vi "DIALOG_Cluster Item Selection.vi"(7 "Action":T4=enum."Bundler Insert", 8 "Error In":errorcluster, 9 "User VI Ref":refnum<vi>, 10 "Affected Items":T2, 11 "Display Items":T3[](array[typedef])) -> (0 "Error Out":errorcluster, 1 "Hide Full Names Out":bool=TRUE, 2 "Action Choice Out":enum32{"Choice 1", "Choice 2"}(radio), 3 "Selected Items (tags)":string[](array[string]))   [LabVIEW 2023]
doc: "Dialog to select items from the input cluster ref. \n\nFilter narrows list of items.\nDown key puts focus on tree and selects first item.\nUp and Down keps navigate tree.\nMultiple items can be selected.\n\nIn case of action \"Delete\" (\"Remove elements(s)...\" selected), list will show all elements currently displayed, else it will show all elements availabel to undle or unbundle.\n\nOutput is a list of the selected item tags.\n\nSelected element is the item clicked in a bundler node, displayed ot help user remember where an insert will happen."
uses:
  controls/Done Button.ctl
  controls/action enum.ctl
  cluster/Cluster Element Description.ctl
  top/BundleMagic.ctl
  utils/Controls/Get-Set Enum.ctl
  LabVIEW-common/String/Select All/String Select All CTRL-A_all string.vi
  <userlib>/_OpenG.lib/appcontrol/appcontrol.llb/openg_application_control.lvlib
  <userlib>/_OpenG.lib/error/error.llb/openg_error.lvlib
  Libraries/Tree Handler/Tree Handlr.lvlib
panel:
  in  "Filter":string
  in  "Tree":string[](tree)
  in  "Hide Full Names":bool=TRUE
  in  "Select Unwired":bool
  out "Selected Element String":string
  in  "Action Choice Radio Buttons":enum32{"Choice 1", "Choice 2"}(radio)
  in  "Done":T1
  out "error out":errorcluster
  in  "Show radio":bool
  in  "C1":T5
  # "All panes scroll to origin at runtime, so we don't have to worry about pane placements\n\nThis pane contracts at runtime and vertical splitter to left sticks to right at runtime so resizing functions happen as expected."
  # "Debug"
  # "Debug Cluster"
  # "(Use for debug if display items empty)"
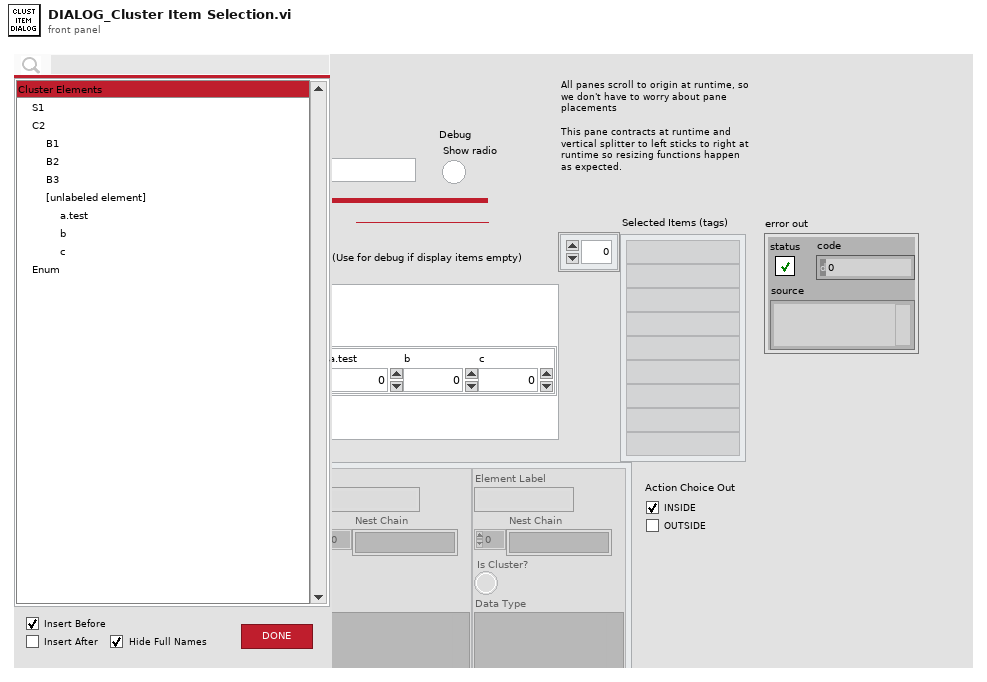
[diagram p1: front panel]
types:
  T1 = typedef "Done Button.ctl" = bool
  T2 = typedef "BundleMagic.ctl" = cluster{"Terminals":refnum<vi>[], "Wires":refnum<vi>[], "Named Bundler":refnum<vi>[], "Named Unbundler":refnum<vi>[], "In Place Cluster Node":refnum<vi>[], "Class Specifier Constant":refnum<vi>[], "Property Node":refnum<vi>[], "Invoke Node":refnum<vi>[], "Refnum Control":refnum<vi>[]}
  T3 = typedef "Cluster Element Description.ctl" = cluster{"Element Label":string, "Nest Chain":string[], "Is Cluster?":bool, "Data Type":variant, "Bundler Label":string, "Disabled":bool, "Unwired":bool, "Tree Tag":string}
  T4 = typedef "action enum.ctl" = enum16{"[NONE]", "APP_SEPARATOR", "Wire Bundle", "Wire Unbundle", "Terminal Unbundle", "Terminal Bundle", "Bundler Move Up", "Bundler Move Down", "Bundler Insert", "Bundler Remove", "Bundler Remove Unwired", "Bundler Reorder", "In Place Insert", "In Place Remove", "In Place Remove Unwired", "In Place Reorder", "Wire Properties", "Wire Method", "Terminal Properties", "Terminal Method", "Property Move Up", "Property Move Down", "Properties Insert", "Properties Remove", "Properties Remove Unwired", "Properties Reorder", "Method Change", "Class For Constant", "Class For Control", "Class For Node", "Class Name to Clipboard"}
  T5 = cluster{"S1":string, "C2":cluster{"B1":bool, "B2":bool, "B3":bool, cluster{"a.test":dbl, "b":i32, "c":u8}}, "Enum":enum16{""}}
  T6 = typedef "Get-Set Enum.ctl" = enum16{"Get", "Set"}
  T7 = typedef "LVPoint32TypeDef.ctl" = cluster{"Horizontal":i32, "Vertical":i32}
  T8 = cluster{"Shift":bool, "Ctrl":bool, "Alt":bool, "Cmd":bool, "Opt":bool}
  T9 = typedef "eventvkey.ctl" = enum16{"ASCII", "Enter", "Return", "Shift", "Ctrl", "Alt", "Cmd", "Opt", "Caps", "NumLock", "Clear", "Break", "Up", "Down", "Left", "Right", "Insert", "Delete", "Home", "End", "PageUp", "PageDown", "Escape", "Help", "Pause", "ScrollLock", "F1", "F2", "F3", "F4", "F5", "F6", "F7", "F8", "F9", "F10", "F11", "F12", "F13", "F14", "F15", "F16", "F17", "F18", "F19", "F20", "F21", "F22", "F23", "F24", "Play", "VolumeUp", "VolumeDown", "Mute", "Two Byte Char"}
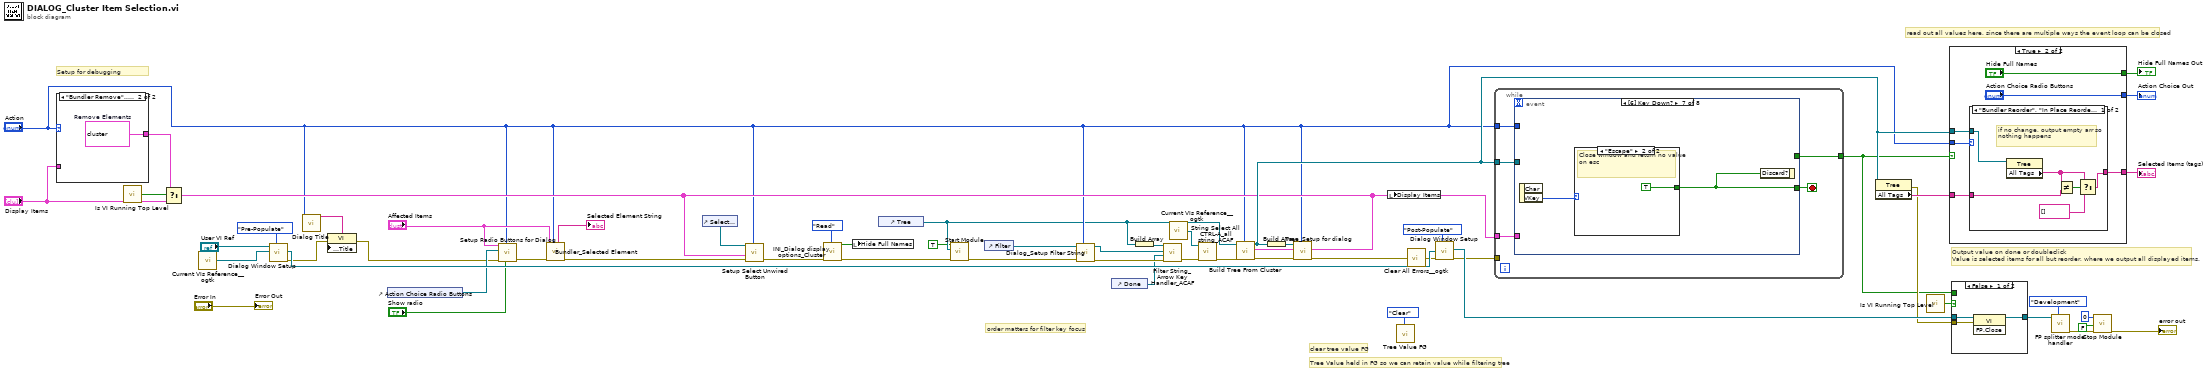
[diagram p0: block diagram]
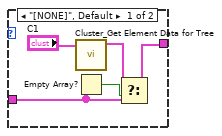
[diagram p2: hidden frame]
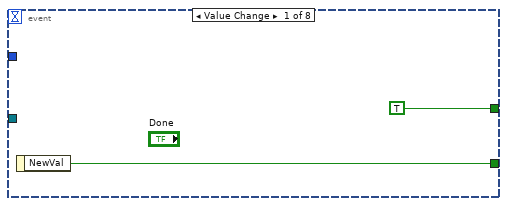
[diagram p3: hidden frame]
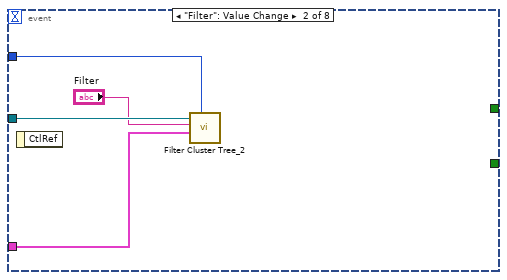
[diagram p4: hidden frame]
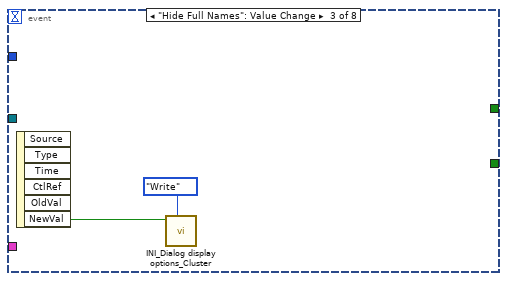
[diagram p5: hidden frame]
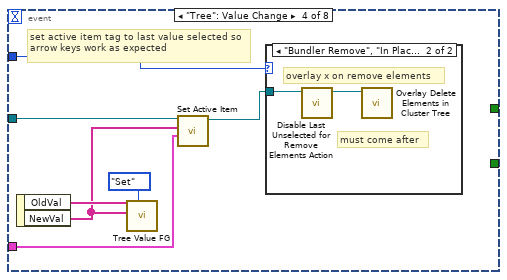
[diagram p6: hidden frame]
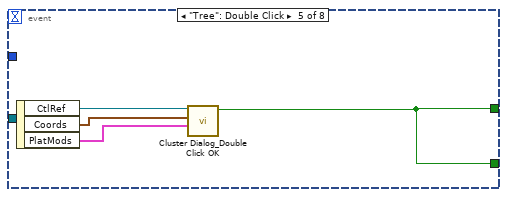
[diagram p8: hidden frame]
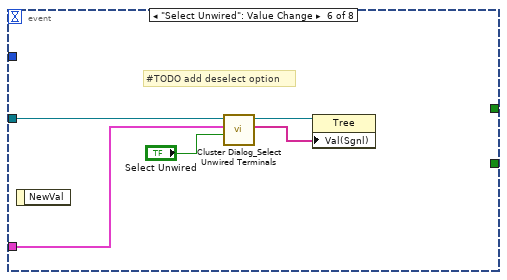
[diagram p9: hidden frame]
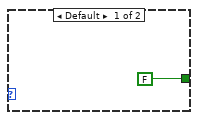
[diagram p10: hidden frame]
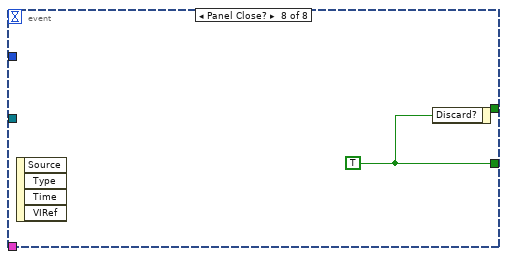
[diagram p11: hidden frame]
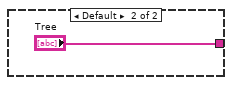
[diagram p13: hidden frame]
diagram:
  # "order matters for filter key focus"
  # "clear tree value FG"
  # "Setup for debugging"
  # "Tree Value held in FG so we can retain value while filtering tree"
  # "read out all values here, since there are multiple ways the event loop can be closed"
  # "Output value on done or doubleclick\nValue is selected items for all but reorder, where we output all displayed items."
  n1 = case shown="\"Bundler Remove\"..\"Bundler Reorder\"" "Action" {
    tunnel: [w61 w63] -> w46
    tunnel: "Display Items" -> [w60 _]
    frame "[NONE]", Default {
      n2 = call "Cluster_Get Element Data for Tree.vi"("Data Type"="C1") -> ("Cluster Element Data Aray"=w62:T3[])  [unwired: 10 in]
      n3 = Empty Array?(array=w60) -> (empty?=w59:bool)
      n4 = Select(t=w62, s=w59, f=w60) -> (s? t:f=w61:T3[])
    }
    frame "Bundler Remove".."Bundler Reorder" {
      w63 = T3[] [{"Element Label"="N1", "Nest Chain"=[], "Is Cluster?"=FALSE, "Data Type"=variant(dbl 0.0), "Bundler Label"="N1", "Disabled"=FALSE, "Unwired"=FALSE, "Tree Tag"="0[$`~g;}N1"}, {"Element Label"="N2", "Nest Chain"=["C1"], "Is Cluster?"=TRUE, "Data Type"=variant(dbl 0.0), "Bundler Label"="C1.N2", "Disabled"=FALSE, "Unwired"=FALSE, "Tree Tag"="C1[$`~g;}C1[$`~g;}N2"}, {"Element Label"="Boolean", "Nest Chain"=["C1"], "Is Cluster?"=TRUE, "Data Type"=variant(bool FALSE), "Bundler Label"="C1.Boolean", "Disabled"=FALSE, "Unwired"=TRUE, "Tree Tag"="C2[$`~g;}C1[$`~g;}Boolean"}, {"Element Label"="C1", "Nest Chain"=[], "Is Cluster?"=FALSE, "Data Type"=variant(cluster{"N2":dbl, "Boolean":bool} {"N2"=0.0, "Boolean"=FALSE}), "Bundler Label"="C1", "Disabled"=FALSE, "Unwired"=FALSE, "Tree Tag"="3[$`~g;}C1"}, {"Element Label"="String", "Nest Chain"=[], "Is Cluster?"=FALSE, "Data Type"=variant(string ""), "Bundler Label"="String", "Disabled"=FALSE, "Unwired"=FALSE, "Tree Tag"="4[$`~g;}String"}]  # Remove Elements
    }
  }
  n5 = call "Is VI Running Top Level.vi"() -> ("Top Level?"=w47:bool)  [unwired: 5 in]
  n6 = Select(t=w46, s=w47, f="Display Items") -> (s? t:f=w19:T3[])
  n7 = call <userlib>:"Current VIs Reference__ogtk.vi"() -> ("Current VI's reference"=w26:refnum<vi>)  [unwired: 5 in]
  n8 = call "Dialog Window Setup.vi"("Action"=enum16{"Pre-Populate", "Post-Populate"}."Pre-Populate", "Dialog VI Ref In [Parent]"=w26, "Align-to Window Ref"="User VI Ref") -> ("error out"=w24:errorcluster, "Dialog VI Ref Out"=w51:refnum<vi>)  [unwired: 7 in]
  n9 = call "Dialog Title.vi"("Action"="Action") -> ("Window Title"=w32:string)  [unwired: 10 in]
  n10 = property class="VI"(error in=w24, "Front Panel.Title"=w32) -> (error out=w23:errorcluster)  [unwired: 1 in, 1 out]
  n11 = control-ref of="Action Choice Radio Buttons"() -> (w34:refnum<vi>)
  n12 = call "Setup Radio Buttons for Dialog.vi"("Show Radio"="Show radio", "Action"="Action", "error in (no error)"=w23, "Action Choice Ref"=w34, "Affected Items"="Affected Items") -> ("error out"=w22:errorcluster)  [unwired: 6 in]
  n13 = call "Bundler_Selected Element.vi"("Action"="Action", "error in (no error)"=w22, "Affected Items"="Affected Items") -> ("error out"=w21:errorcluster, "Display String"=→"Selected Element String":string)  [unwired: 2 in, 5 out]
  n14 = control-ref of="Select Unwired"() -> (w33:refnum<vi>)
  n15 = call "Setup Select Unwired Button.vi"("Action"="Action", "error in (no error)"=w21, "Display Items"=w19, "Boolean in"=w33) -> ("error out"=w11:errorcluster)  [unwired: 7 in]
  n16 = call "INI_Dialog display options_Cluster.vi"("File Action"=enum16{"Read", "Write"}."Read", "error in (no error)"=w11) -> ("error out"=w6:errorcluster, "Hide Full Names Out"=w10:bool)  [unwired: 8 in]
  n17 = local write "Hide Full Names"(w10) -> ()
  n18 = control-ref of="Tree"() -> (w4:refnum<vi>)
  n19 = call "Start Module.vi"("error in"=w6, "Tree Ref"=w4, "Run as Singleton? (F)"=TRUE) -> ("error out"=w5:errorcluster)  [unwired: 5 in, 3 out]
  n20 = control-ref of="Filter"() -> (w27:refnum<vi>)
  n21 = call "Dialog_Setup Filter String.vi"("Action"="Action", "error in"=w5, "Filter String Ref"=w27) -> ("error out"=w18:errorcluster, "Filter String Ref Out"=w14:refnum<vi>)  [unwired: 7 in]
  n22 = control-ref of="Done"() -> (w16:refnum<vi>)
  n23 = Build Array(w4) -> (w15:refnum<vi>[])
  n24 = call "Filter String_Arrow Key Handler_ACAF.vi"("error in (no error)"=w18, "Done Ref"=w16, "Filter String Ref"=w14, "Tree Ref Array"=w15) -> ("error out"=w17:errorcluster)  [unwired: 7 in]
  n25 = call <userlib>:"Current VIs Reference__ogtk.vi"() -> ("Current VI's reference"=w25:refnum<vi>)  [unwired: 5 in]
  n26 = call "String Select All CTRL-A_all string_ACAF.vi"("error in (no error)"=w17, "VI Ref"=w25) -> ("error out"=w42:errorcluster)  [unwired: 9 in]
  n27 = call "Build Tree From Cluster.vi"("Action"="Action", "error in"=w42, "Display Items"=w19, "Tree Ref"=w4) -> ("error out"=w41:errorcluster, "Tree Ref Out"=w48:refnum<vi>)  [unwired: 6 in]
  n28 = Build Array(w48) -> (w40:refnum<vi>[])
  n29 = call "Tree_Setup for dialog.vi"("Action"="Action", "error in"=w41, "Tree Ref"=w40) -> ("error out"=w39:errorcluster)  [unwired: 7 in, 1 out]
  n30 = local write "Display Items"(w19) -> ()
  n31 = call "Tree Value FG.vi"("Get Set Enum"=enum16{"Get", "Set", "Clear"}."Clear") -> ()  [unwired: 10 in, 1 out]
  n32 = call <userlib>:"Clear All Errors__ogtk.vi"("Error In"=w39) -> ("Error Out"=w37:errorcluster)  [unwired: 3 in]
  n33 = call "Dialog Window Setup.vi"("Action"=enum16{"Pre-Populate", "Post-Populate"}."Post-Populate", "error in"=w37, "Dialog VI Ref In [Parent]"=w51) -> ("error out"=w49:errorcluster, "Dialog VI Ref Out"=w50:refnum<vi>)  [unwired: 7 in]
  n34 = while {
    tunnel: w48 -> [w67]
    tunnel: [w66] -> w43
    tunnel: "Action" -> [w65]
    tunnel: w19 -> [w64]
    tunnel: w49 -> [_]
    stop <- w68 stop-if-true
    n35 = event shown="[6] Key Down?" {
      selector: _ -> [_ _ _ _ _ _ _ _]
      dyn-events: _ -> [_ _ _ _ _ _ _ _]
      timeout: _ -> [_ _ _ _ _ _ _ _]
      tunnel: [w70 _ _ _ w89 _ w95 w99] -> w68
      tunnel: w67 -> [_ w74 _ w81 _ w93 _ _]
      tunnel: [TRUE _ _ _ w89 _ _ _] -> w66
      tunnel: w65 -> [_ w71 _ w83 _ _ _ _]
      tunnel: w64 -> [_ w72 _ w77 _ w94 _ _]
      event Value Change {
        n36 = event-data() -> ("NewVal"=w70:T1)  [unwired: 1 in]
      }
      event "Filter": Value Change {
        n37 = event-data() -> ()  [unwired: 1 in, 1 out]
        n38 = call "Filter Cluster Tree_2.vi"("Action"=w71, "Display Items"=w72, "Filter Str"="Filter", "Tree Ref"=w74) -> ()  [unwired: 7 in, 1 out]
      }
      event "Hide Full Names": Value Change {
        n39 = event-data() -> ("NewVal"=w75:bool)  [unwired: 1 in, 5 out]
        n40 = call "INI_Dialog display options_Cluster.vi"("File Action"=enum16{"Read", "Write"}."Write", "Hide Full Names"=w75) -> ()  [unwired: 8 in, 2 out]
      }
      event "Tree": Value Change {
        # "set active item tag to last value selected so arrow keys work as expected"
        n41 = event-data() -> ("OldVal"=w80:string[], "NewVal"=w78:string[])  [unwired: 1 in]
        n42 = call "Tree Value FG.vi"("Get Set Enum"=Get-Set_Enum."Set", "NewVal"=w78, "Old Val"=w80) -> ()  [unwired: 8 in, 1 out]
        n43 = call "Set Active Item.vi"("Display Items"=w77, "NewVal"=w78, "TreeControl in"=w81) -> ("TreeControl out"=w82:refnum<vi>)  [unwired: 8 in]
        n44 = case shown="\"Bundler Remove\", \"In Place Remove\"" w83 {
          tunnel: w82 -> [_ w85]
          frame "[NONE]", Default {
          }
          frame "Bundler Remove", "In Place Remove" {
            # "overlay x on remove elements"
            # "must come after"
            n45 = call "Disable Last Unselected for Remove Elements Action.vi"("Tree Ref"=w85) -> ("Tree Ref Out"=w84:refnum<vi>)  [unwired: 8 in, 2 out]
            n46 = call "Overlay Delete Elements in Cluster Tree.vi"("Tree Ref"=w84) -> ()  [unwired: 10 in, 1 out]
          }
        }
      }
      event "Tree": Double Click {
        # "Double click to select and end entry"
        n47 = event-data() -> ("CtlRef"=w88:refnum<vi>, "Coords"=w87:T7, "PlatMods"=w86:T8)  [unwired: 1 in]
        n48 = call "Cluster Dialog_Double Click OK.vi"("PlatMods"=w86, "Coords"=w87, "TreeControl in"=w88) -> ("Valid Item Double Clicked"=w89:bool)  [unwired: 8 in]
      }
      event "Select Unwired": Value Change {
        # "#TODO add deselect option"
        n49 = event-data() -> ()  [unwired: 1 in, 1 out]
        n50 = call "Cluster Dialog_Select Unwired Terminals.vi"("Select Unwired"="Select Unwired", "Display Items"=w94, "Tree Ref"=w93) -> ("Selected items"=w90:string[], "Tree Ref Out"=w91:refnum<vi>)  [unwired: 7 in]
        n51 = property class="Tree"(reference=w91, "Val(Sgnl)"=w90) -> ()  [unwired: 1 in, 2 out]
      }
      event Key Down? {
        # "Quit on escape"
        n52 = event-data() -> ("VKey"=w96:T9)  [unwired: 1 in, 1 out]
        n53 = case shown="\"Escape\"" w96 {
          tunnel: [FALSE TRUE] -> w95
          frame Default {
          }
          frame "Escape" {
            # "Close window and return no value on esc"
          }
        }
        n54 = event-data("Discard?"=w95) -> ()  [unwired: 1 in, 1 out]
      }
      event Panel Close? {
        w99 = TRUE
        # "close and return no value on panel close"
        n55 = event-data() -> ()  [unwired: 1 in, 4 out]
        n56 = event-data("Discard?"=w99) -> ()  [unwired: 1 in, 1 out]
      }
    }
  }
  n57 = property class="Tree"(reference=w48) -> (error out=w44:errorcluster, "All Tags"=w52:string[])  [unwired: 1 in, 1 out]
  n58 = call "Is VI Running Top Level.vi"() -> ("Top Level?"=w54:bool)  [unwired: 5 in]
  n59 = case shown="True" w43 {
    tunnel: [_ w105] -> w57
    tunnel: "Action" -> [_ w104]
    tunnel: w48 -> [_ w103]
    tunnel: [_ "Action Choice Radio Buttons"] -> w55
    tunnel: w52 -> [_ w101]
    tunnel: [_ "Hide Full Names"] -> w9
    frame False {
    }
    frame True {
      n60 = case shown="\"Bundler Reorder\", \"In Place Reorder\"" w104 {
        tunnel: [w106 "Tree"] -> w105
        tunnel: w103 -> [w111 _]
        tunnel: w101 -> [w110 _]
        frame "Bundler Reorder", "In Place Reorder" {
          # "if no change, output empty arr so nothing happens"
          n61 = property class="Tree"(reference=w111) -> ("All Tags"=w107:string[])  [unwired: 1 in, 2 out]
          n62 = Not Equal?(x=w107, y=w110) -> (x != y?=w109:bool)
          n63 = Select(t=w107, s=w109, f=string[] []) -> (s? t:f=w106:string[])
        }
        frame Default {
        }
      }
    }
  }
  "Selected Items (tags)" <- w57
  "Action Choice Out" <- w55
  "Hide Full Names Out" <- w9
  n64 = case shown="False" w54 {
    tunnel: w50 -> [w115 w116]
    tunnel: [w114 w116] -> w53
    tunnel: w44 -> [w113 _]
    tunnel: w43 -> [_ _]
    frame False {
      n65 = invoke class="VI" method="FP.Close"(reference=w115, error in=w113) -> (reference out=w114:refnum<vi>)  [unwired: 1 in, 2 out]
    }
    frame True {
    }
  }
  n66 = call "FP splitter mode handler.vi"("Mode"=enum16{"Run", "Development"}."Development", "VI Ref In"=w53) -> ("error out"=w8:errorcluster)  [unwired: 8 in, 1 out]
  n67 = call "Stop Module.vi"("error in"=w8, "Wait for Module to stop? (F)"=FALSE, "Module ID"=0) -> ("error out"=→"error out":errorcluster)  [unwired: 8 in]
  "Error Out" <- "Error In"
